vi "CRC16 - PS.vi"(11 "要校验的字符串（十六进制显示）":string) -> (2 "连接的字符串(16进制)":string, 3 "CRC16先低后高":string)   [LabVIEW 2026, in "UI-压力.lvlib" / "Acquisition.lvlib"]
uses:
  Acquisition.lvlib
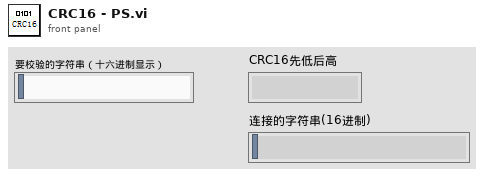
[diagram p1: front panel]
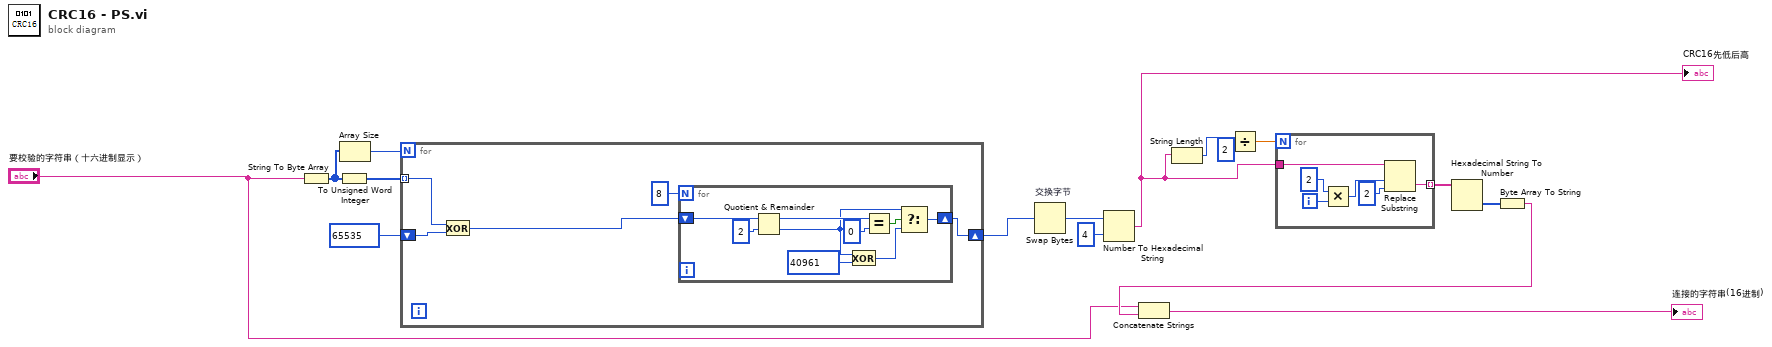
[diagram p0: block diagram]
diagram:
  n1 = String To Byte Array(string="要校验的字符串（十六进制显示）") -> (unsigned byte array=w1:u8[])
  n2 = To Unsigned Word Integer(number=w1) -> (unsigned 16bit integer=w2:u16[])
  n3 = Array Size(array=w1) -> (size(s)=w3:i32)
  n4 = for {
    N: w3 -> [_]
    tunnel: w2 -> [w21] mode=indexing
    shift-right: [w18] -> w5
    shift-left: u16 65535 ("y") -> [w19]
    n5 = Exclusive Or(1:w19, 2:w21) -> (0:w17:u16)
    n6 = for {
      N: 8 -> [_]
      shift-right: [w22] -> w18
      shift-left: w17 -> [w23]
      n7 = Quotient & Remainder(x=w23, y=u16 2) -> (x-y*floor(x/y)=w29:u16, floor(x/y)=w26:u16)
      n8 = Exclusive Or(1:u16 40961 ("y"), 2:w26) -> (0:w24:u16)
      n9 = Equal?(x=w29, y=u16 0) -> (x = y?=w27:bool)
      n10 = Select(t=w26, s=w27, f=w24) -> (s? t:f=w22:u16)
    }
  }
  n11 = Swap Bytes "交换字节"(anything=w5) -> (byte swapped=w6:u16)
  n12 = Number To Hexadecimal String(1:i16 4 ("宽度(-)"), 2:w6) -> (0:w16:string)
  "CRC16先低后高" <- w16
  n13 = String Length(string=w16) -> (length=w10:i32)
  n14 = Divide(x=w10, y=2) -> (x/y=w12:dbl)
  n15 = for {
    N: w12 -> [_]
    tunnel: w16 -> [w32]
    tunnel: [w31] -> w13 mode=indexing
    i -> [w36]
    n16 = Multiply(x=2, y=w36) -> (x*y=w34:i32)
    n17 = Replace Substring(2:2 ("长度（子字符串长度）"), 3:w34, 5:w32) -> (0:w31:string)  [unwired: 1 in, 1 out]
  }
  n18 = Hexadecimal String To Number(string=w13) -> (number=w14:u32[])  [unwired: 2 in, 1 out]
  n19 = Byte Array To String(unsigned byte array=w14) -> (string=w15:string)
  n20 = Concatenate Strings("要校验的字符串（十六进制显示）", w15) -> (→"连接的字符串(16进制)":string)
